vi "gen scan waveforms - virtual.vi"(0 "overshoot time (ms) (applied twice)":dbl=0.01, 4 "Scanner calibration":cluster{"Offset":dbl, "Amplitude":dbl}[](array[cluster])=[{"Offset"=2.5, "Amplitude"=-0.31}, {"Offset"=2.5, "Amplitude"=0.2}, {"Offset"=2.5, "Amplitude"=0.0}, {"Offset"=2.5, "Amplitude"=0.0}] {"Amplitude" min=-5.0 max=5.0 step=0.005; "Offset" min=0.0 max=5.0 step=0.005}, 6 "Signal delays":T2={"ETL delay (samples)"=10, "Scanner delay (samples)"=-25, "Laser delay (samples)"=2}, 7 "Z Slices":cluster{"start":dbl, "delta":dbl, "end":dbl}={"start"=100.0, "delta"=-1.355, "end"=20.0}, 8 "AO sample rate":dbl=100000.0 format="%.2p", 9 "Flash duration (s)":dbl, 10 "frame period (s)":dbl=0.006, 11 "volume period (s)":dbl) -> (1 "Digital signals":u8[][](array[numeric]), 2 "Analog signals":dbl[][](array[numeric]))   [LabVIEW 2020, in "Scan Generators.lvlib"]
uses:
  Scan Generators.lvlib
  <vilib>/Analysis/baseanly.llb/Scale 1D.vi
  <vilib>/Analysis/1siggen.llb/Ramp Pattern by Delta.vi
  <vilib>/Waveform/DWDTOps.llb/DWDT Boolean Array to Digital.vi
  <vilib>/Analysis/NI_AALBase.lvlib
panel:
  out "Reset time":dbl
  out "Mixed Signal Graph":T1(graph)
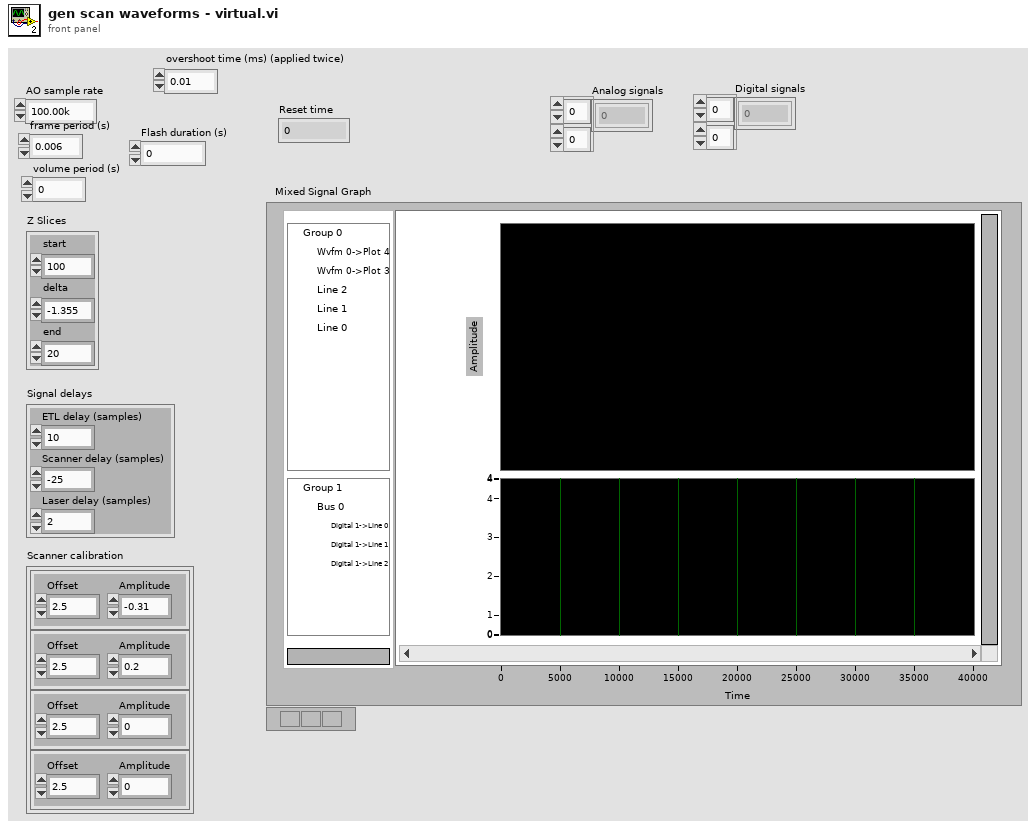
[diagram p1: front panel]
types:
  T1 = cluster{"Analog Waveforms 2":dbl[][], "digital waveform":digitalwaveform}
  T2 = cluster{"ETL delay (samples)":i32, "Scanner delay (samples)":i32, "Laser delay (samples)":i32}
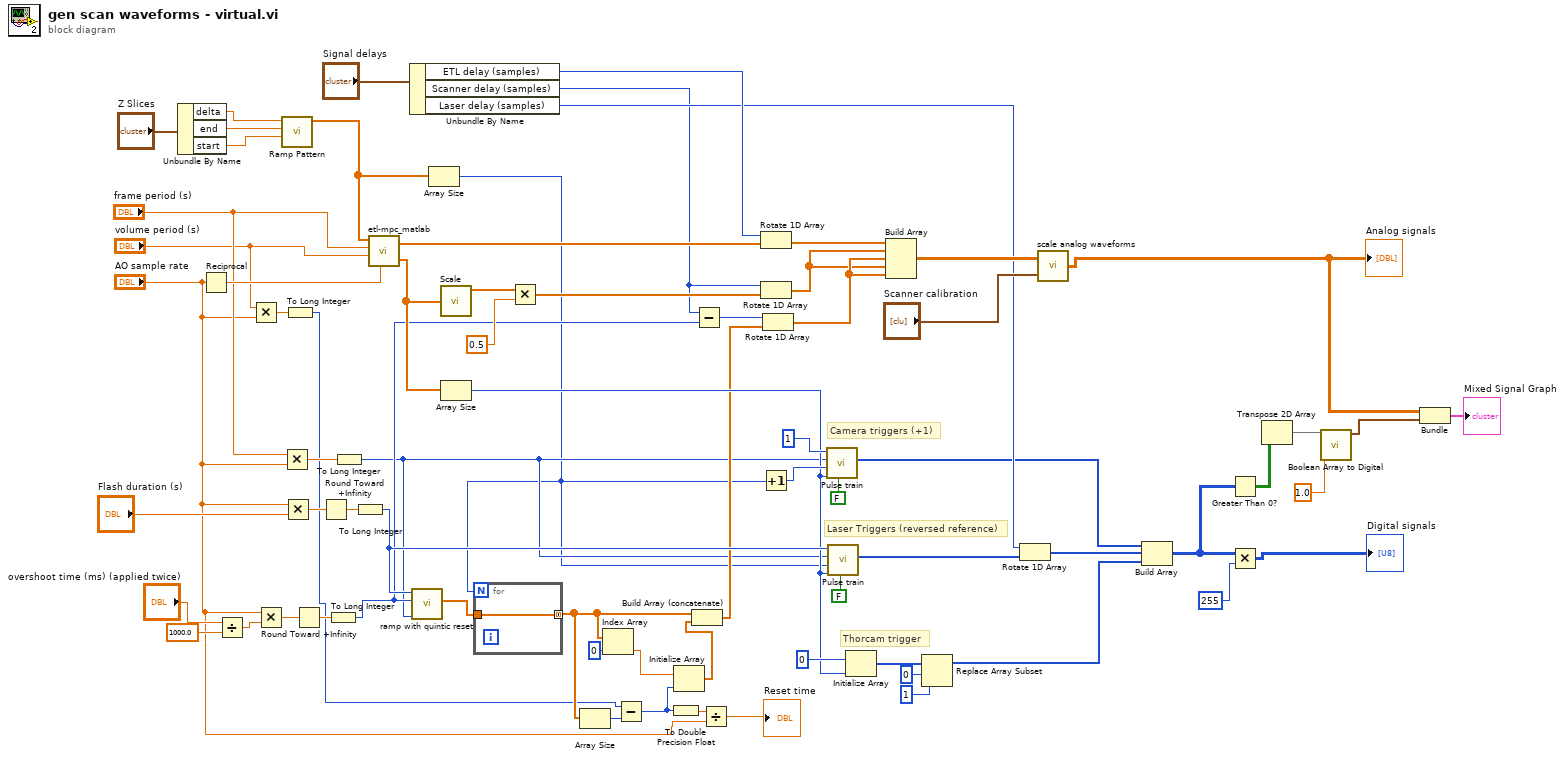
[diagram p0: block diagram]
diagram:
  # "Thorcam trigger"
  # "Laser Triggers (reversed reference)"
  # "Camera triggers (+1)"
  n1 = Unbundle By Name("Z Slices") -> ("delta"=w62:dbl, "end"=w63:dbl, "start"=w64:dbl)
  n2 = Reciprocal(x="AO sample rate") -> (1/x=w61:dbl)
  n3 = Divide(x="overshoot time (ms) (applied twice)", y=1000.0) -> (x/y=w20:dbl)
  n4 = Multiply(x="volume period (s)", y="AO sample rate") -> (x*y=w14:dbl)
  n5 = Multiply(x="AO sample rate", y=w20) -> (x*y=w27:dbl)
  n6 = call-poly <vilib>:"Ramp Pattern.vi"("start"=w64, "end"=w63, "delta"=w62) -> ("Ramp Pattern"=w44:dbl[])  [unwired: 6 in, 2 out]
  n7 = Multiply(x="frame period (s)", y="AO sample rate") -> (x*y=w45:dbl)
  n8 = Multiply(x="AO sample rate", y="Flash duration (s)") -> (x*y=w49:dbl)
  n9 = To Long Integer(number=w14) -> (32bit integer=w5:i32)
  n10 = Round Toward +Infinity(x=w27) -> (ceil(x): smallest int >= x=w26:dbl)
  n11 = Round Toward +Infinity(x=w49) -> (ceil(x): smallest int >= x=w48:dbl)
  n12 = To Long Integer(number=w26) -> (32bit integer=w23:i32)
  n13 = To Long Integer(number=w45) -> (32bit integer=w12:i32)
  n14 = To Long Integer(number=w48) -> (32bit integer=w28:i32)
  n15 = call "etl-mpc_matlab.vi"("AO Sample Period"=w61, "volume period"="volume period (s)", "frame period"="frame period (s)", "slice array"=w44) -> ("Predicted Scan Path"=w43:dbl[], "ETL scan waveform"=w56:dbl[])  [unwired: 2 in]
  n16 = Unbundle By Name("Signal delays") -> ("ETL delay (samples)"=w55:i32, "Scanner delay (samples)"=w25:i32, "Laser delay (samples)"=w40:i32)
  n17 = call "ramp with quintic reset.vi"("Frame Samples"=w12, "Overshoot Samples"=w23, "Ramp Samples"=w28) -> ("Scan waveform"=w18:dbl[])  [unwired: 8 in]
  n18 = Array Size(array=w44) -> (size(s)=w10:i32)
  n19 = call-poly <vilib>:"Scale.vi"("X"=w43) -> ("Y=(X-offset)/scale"=w60:dbl[])  [unwired: 3 out]
  n20 = Array Size(array=w43) -> (size(s)=w19:i32)
  n21 = for {
    N: w10 -> [_]
    tunnel: w18 -> [w72]
    tunnel: [w72] -> w7 mode=concatenating
  }
  n22 = Multiply(x=w60, y=0.5) -> (x*y=w57:dbl[])
  n23 = Array Size(array=w7) -> (size(s)=w6:i32)
  n24 = Index Array(array=w7, index=0) -> (element=w15:dbl)
  n25 = Subtract(x=w5, y=w6) -> (x-y=w4:i32)
  n26 = To Double Precision Float(number=w4) -> (double precision float=w3:dbl)
  n27 = Initialize Array(w15, w4) -> (w11:dbl[])
  n28 = Build Array (concatenate)(w7, w11) -> (w17:dbl[])
  n29 = Subtract(x=w25, y=w23) -> (x-y=w24:i32)
  n30 = Divide(x=w3, y="AO sample rate") -> (x/y=→"Reset time":dbl)
  n31 = Rotate 1D Array(1:w56, 2:w55) -> (0:w54:dbl[])
  n32 = Rotate 1D Array(1:w57, 2:w25) -> (0:w8:dbl[])
  n33 = Increment(x=w10) -> (x+1=w42:i32)
  n34 = Rotate 1D Array(1:w17, 2:w24) -> (0:w9:dbl[])
  n35 = call "Pulse train.vi"("Reverse?"=FALSE, "Total length"=w19, "Cycles"=w42, "Cycle length"=w12, "Pulse length"=1) -> ("output array"=w33:u8[])  [unwired: 6 in]
  n36 = call "Pulse train.vi"("Reverse?"=FALSE, "Total length"=w19, "Cycles"=w10, "Cycle length"=w12, "Pulse length"=w28) -> ("output array"=w41:u8[])  [unwired: 6 in]
  n37 = Initialize Array(u8 0 ("element"), w19) -> (w37:u8[])
  n38 = Build Array(w54, w8, w9, w8, w9) -> (w53:dbl[][])
  n39 = Replace Array Subset(array=w37, new element=u8 1 ("new element/subarray"), index=0) -> (w32:u8[])
  n40 = Rotate 1D Array(1:w41, 2:w40) -> (0:w34:u8[])
  n41 = call "scale analog waveforms.vi"("Scaling parameters"="Scanner calibration", "Analog Waveforms"=w53) -> ("Analog Waveforms 2"=w67:dbl[][])
  "Analog signals" <- w67
  n42 = Build Array(w33, w34, w32) -> (w31:u8[][])
  n43 = Greater Than 0?(x=w31) -> (x > 0?=w70:bool[][])
  n44 = Multiply(x=w31, y=u8 255) -> (x*y=→"Digital signals":u8[][])
  n45 = Transpose 2D Array(2D array=w70) -> (transposed array=w69:bool[][])
  n46 = call-poly <vilib>:"Boolean Array to Digital.vi"("sample rate"=1.0, "boolean array"=w69) -> ("digital waveform"=w66:digitalwaveform)  [unwired: 8 in, 1 out]
  n47 = Bundle("Analog Waveforms 2"=w67, "digital waveform"=w66) -> (→"Mixed Signal Graph":T1)  [unwired: 1 in]
